vi "Periodic Tasks.vi"(8 "error in":errorcluster) -> ()   [LabVIEW 2018]
doc: "This VI runs in parallel to other tasks. It can contain as many user-defined periodic loops as you need. These can carry out PID or other sorts of timed response."
uses:
  <vilib>/Rock Robotics/WPI/DriverStation/WPI_DriverStationRobotMode2.ctl
  <vilib>/Rock Robotics/WPI/Utilities/WPI_GetSetVariantRefNum.vi
  Robot Global Data.vi
  <vilib>/Rock Robotics/WPI/ThirdParty/Phoenix-LabVIEW/Motor Controller/Get/CTRE_Phoenix_MotorController_GetSelectedSensorData.vi
panel:
  out "Y position":dbl
  out "X position":dbl
  out "status":dbl
  out "Yaw":dbl
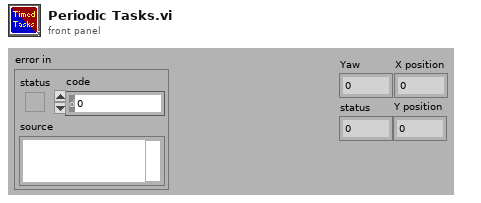
[diagram p1: front panel]
types:
  T1 = typedef "WPI_JoystickDevRef.ctl" = cluster{"Device":T2}
  T2 = typedef "WPI_JoystickDeviceEnum.ctl" = enum16{"USB 0", "USB 1", "USB 2", "USB 3", "USB 4", "USB 5"}
  T3 = typedef "WPI_RobotDriveDevRef.ctl" = cluster{"DevStatus":errorcluster, "Motors[]":T4[], "Square Inputs":bool, "Max Output":dbl}
  T4 = typedef "WPI_MotorControlDeviceRef.ctl" = cluster{"DeviceStatus":errorcluster, "Type":T5, "PWM":cluster{"PWM Channel":T6, "DeadBand":T7}, "CAN":cluster{"Device Number":u8, "SetOutput VI Ref":variant, "GetOutput VI Ref":variant, "Enable VI Ref":variant, "Disable VI Ref":variant, "Data":variant}, "Invert":bool, "DIO PWM":cluster{"PWM \"Enable\" Channel":T6, "DIOChannel":T8, "PWM Rate":dbl}}
  T5 = typedef "WPI_MotorControlType.ctl" = enum16{"PWM", "CAN", "DIO PWM"}
  T6 = typedef "FPGA_DIOPWMChannel.ctl" = enum8{"PWM 0", "PWM 1", "PWM 2", "PWM 3", "PWM 4", "PWM 5", "PWM 6", "PWM 7", "PWM 8", "PWM 9", "PWM MXP 0", "PWM MXP 1", "PWM MXP 2", "PWM MXP 3", "PWM MXP 4", "PWM MXP 5", "PWM MXP 6", "PWM MXP 7", "PWM MXP 8", "PWM MXP 9", "Invalid"}
  T7 = typedef "WPI_PWMDeadband.ctl" = cluster{"Name":string, "maxPositivePwm":i32, "minPositivePwm":i32, "centerPwm":i32, "maxNegativePwm":i32, "minNegativePwm":i32, "angularRange":u16}
  T8 = typedef "FPGA_DIOChannel.ctl" = enum8{"DIO 0", "DIO 1", "DIO 2", "DIO 3", "DIO 4", "DIO 5", "DIO 6", "DIO 7", "DIO 8", "DIO 9", "DIO MXP 0", "DIO MXP 1", "DIO MXP 2", "DIO MXP 3", "DIO MXP 4", "DIO MXP 5", "DIO MXP 6", "DIO MXP 7", "DIO MXP 8", "DIO MXP 9", "DIO MXP 10", "DIO MXP 11", "DIO MXP 12", "DIO MXP 13", "DIO MXP 14", "DIO MXP 15", "SPI Port CS1", "SPI Port CS2", "SPI Port CS3", "SPI Port MISO", "SPI Port MOSI", "Invalid"}
  T9 = cluster{"JoystickDevRef":T1, "RobotDriveDevRef":T3}
  T10 = typedef "WPI_DriverStationRobotMode2.ctl" = enum16{"Autonomous Disabled", "Autonomous Enabled", "Teleop Disabled", "Teleop Enabled", "Disconnected", "Finish", "Test Disabled", "Test Enabled", "Emergency Stopped"}
  T11 = cluster{"Yaw":dbl, "Roll":dbl, "Pitch":dbl, "Heading":dbl, "Fused Heading":dbl}
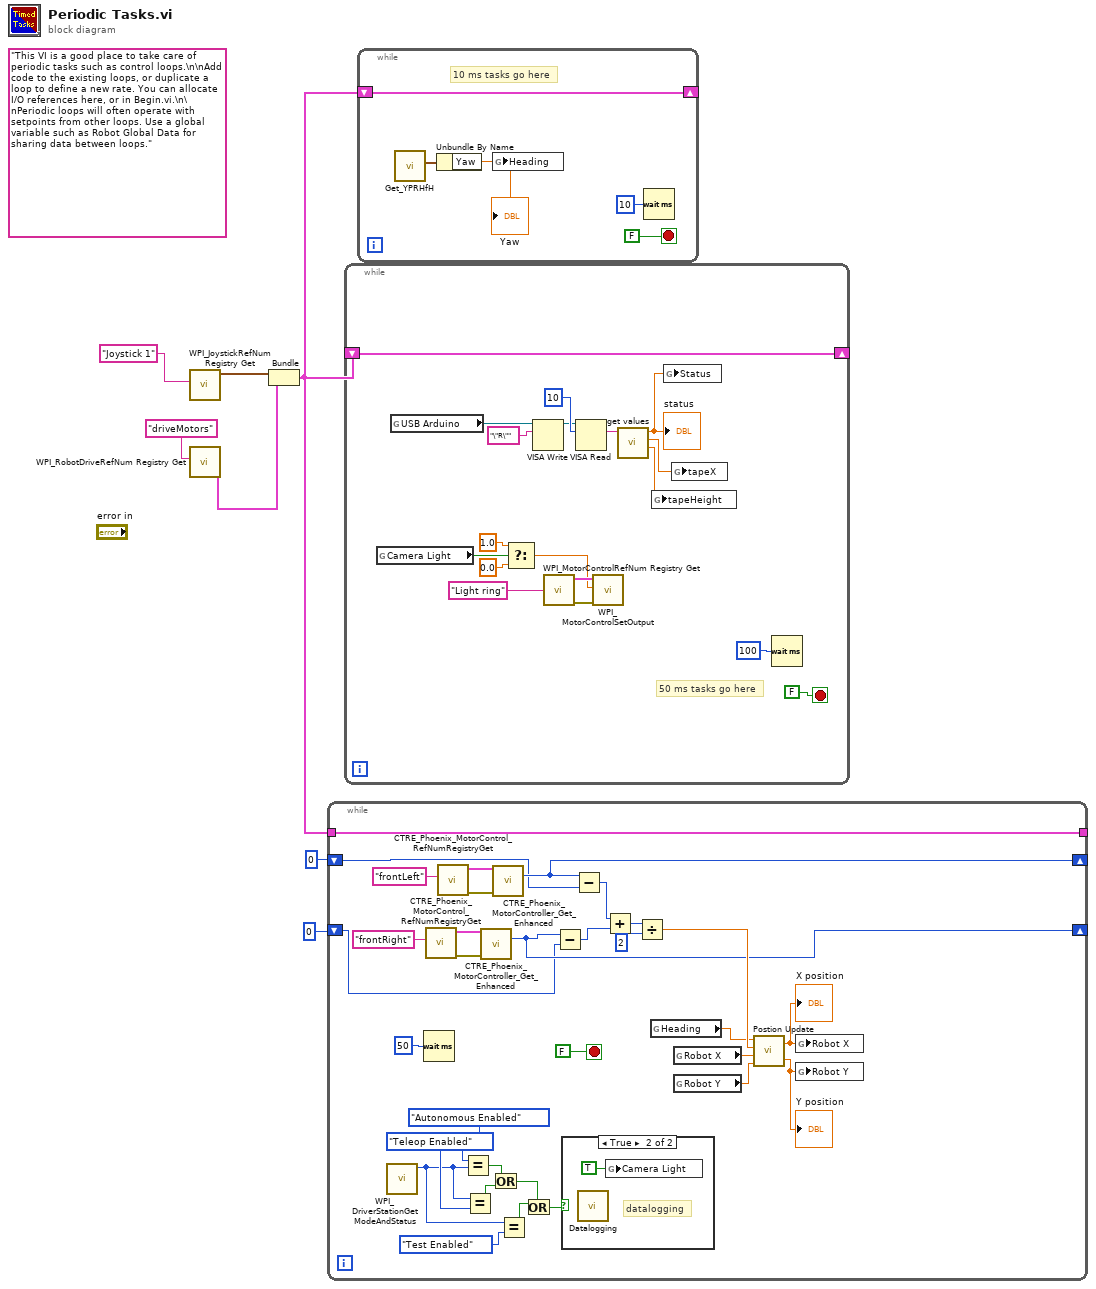
[diagram p0: block diagram]
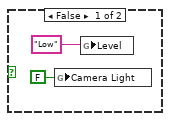
[diagram p2: hidden frame]
diagram:
  (unwired) "This VI is a good place to take care of periodic tasks such as control loops.\n\nAdd code to the existing loops, or duplicate a loop to define a new rate. You can allocate I/O references here, or in Begin.vi.\n\nPeriodic loops will often operate with setpoints from other loops. Use a global variable such as Robot Global Data for sharing data between loops."
  n1 = call <vilib>:"WPI_JoystickRefNum Registry Get.vi"("refnum name"="Joystick 1") -> ("JoystickDevRef"=w5:T1)  [unwired: 1 in, 9 out]
  n2 = call <vilib>:"WPI_RobotDriveRefNum Registry Get.vi"("refnum name"="driveMotors") -> ("RobotDriveDevRef"=w4:T3)  [unwired: 1 in, 9 out]
  n3 = Bundle("JoystickDevRef"=w5, "RobotDriveDevRef"=w4) -> (w3:T9)  [unwired: 1 out]
  n4 = while {
    tunnel: w3 -> [w39]
    tunnel: [w39] -> _
    shift-right: [w22] -> _
    shift-left: 0 -> [w21]
    shift-right: [w20] -> _
    shift-left: 0 -> [w19]
    stop <- FALSE stop-if-true
    n5 = call <vilib>:"WPI_DriverStationGetModeAndStatus.vi"() -> ("Robot Mode"=w12:T10)  [unwired: 10 in, 1 out]
    n6 = Wait (ms)(milliseconds to wait=u32 50) -> ()  [unwired: 1 out]
    n7 = call <vilib>:"CTRE_Phoenix_MotorControl_RefNumRegistryGet.vi"("refnum name"="frontRight") -> ("error out"=w33:errorcluster, "PhoenixMotorControlDevRef"=w31:T4)  [unwired: 9 in]
    n8 = call <vilib>:"CTRE_Phoenix_MotorControl_RefNumRegistryGet.vi"("refnum name"="frontLeft") -> ("error out"=w35:errorcluster, "PhoenixMotorControlDevRef"=w36:T4)  [unwired: 9 in]
    n9 = Equal?(x=WPI_DriverStationRobotMode2."Autonomous Enabled" ("Robot Mode"), y=w12) -> (x = y?=w15:bool)
    n10 = Equal?(x=w12, y=WPI_DriverStationRobotMode2."Teleop Enabled" ("Robot Mode")) -> (x = y?=w9:bool)
    n11 = call-poly <vilib>:"CTRE_Phoenix_MotorController_Get_Enhanced.vi"("PhoenixMotorControlDevRef"=w31, "error in"=w33) -> ("Position (Raw Sensor Units)"=w20:i32)  [unwired: 10 in, 3 out]
    n12 = Or(x=w15, y=w9) -> (x .or. y?=w8:bool)
    n13 = call-poly <vilib>:"CTRE_Phoenix_MotorController_Get_Enhanced.vi"("PhoenixMotorControlDevRef"=w36, "error in"=w35) -> ("Position (Raw Sensor Units)"=w22:i32)  [unwired: 10 in, 3 out]
    n14 = Equal?(x=w12, y=WPI_DriverStationRobotMode2."Test Enabled" ("Robot Mode")) -> (x = y?=w13:bool)
    n15 = Or(x=w13, y=w8) -> (x .or. y?=w10:bool)
    n16 = Subtract(x=w20, y=w19) -> (x-y=w24:i32)
    n17 = case shown="True" w10 {
      frame False {
        n18 = global write "Robot Global Data.vi" "Camera Light"(FALSE ("Camera Light")) -> ()
        n19 = global write "Robot Global Data.vi" "Level"("Low" ("Level")) -> ()
      }
      frame True {
        # "datalogging"
        n20 = call "Datalogging.vi"() -> ()  [unwired: 12 in]
        n21 = global write "Robot Global Data.vi" "Camera Light"(TRUE ("Camera Light")) -> ()
      }
    }
    n22 = Subtract(x=w22, y=w21) -> (x-y=w23:i32)
    n23 = Add(x=w23, y=w24) -> (x+y=w30:i32)
    n24 = Divide(x=w30, y=2) -> (x/y=w28:dbl)
    n25 = global read "Robot Global Data.vi" "Heading"() -> (w27:dbl)
    n26 = global read "Robot Global Data.vi" "Robot X"() -> (w37:dbl)
    n27 = global read "Robot Global Data.vi" "Robot Y"() -> (w38:dbl)
    n28 = call "Postion Update.vi"("Y position in"=w38, "X position in"=w37, "Distance"=w28, "Heading"=w27) -> ("Y position"=w17:dbl, "X position"=w18:dbl)
    "X position" <- w18
    "Y position" <- w17
    n29 = global write "Robot Global Data.vi" "Robot X"(w18) -> ()
    n30 = global write "Robot Global Data.vi" "Robot Y"(w17) -> ()
  }
  n31 = while {
    shift-right: [w58] -> _
    shift-left: w3 -> [w58]
    stop <- FALSE stop-if-true
    # "50 ms tasks go here"
    n32 = global read "Robot Global Data.vi" "Camera Light"() -> (w47:bool)
    n33 = global read "Robot Global Data.vi" "USB Arduino"() -> (w52:refnum<visa-resource-name>)
    n34 = Select(t=1.0, s=w47, f=0.0) -> (s? t:f=w44:dbl)
    n35 = VISA Write(VISA resource name=w52, write buffer="\"R\"") -> (VISA resource name out=w51:refnum<visa-resource-name>)  [unwired: 1 in, 2 out]
    n36 = call <vilib>:"WPI_MotorControlRefNum Registry Get.vi"("refnum name"="Light ring") -> ("error out"=w49:errorcluster, "MotorControlDevRef"=w48:T4)  [unwired: 9 in]
    n37 = VISA Read(VISA resource name=w51, byte count=u32 10) -> (read buffer=w54:string)  [unwired: 1 in, 3 out]
    n38 = call <vilib>:"WPI_MotorControlSetOutput.vi"("error in (no error)"=w49, "Output"=w44, "MotorControlDevRef"=w48) -> ()  [unwired: 6 in, 3 out]
    n39 = call "get values.vi"("USB In"=w54) -> ("insidex (0-319)"=w55:dbl, "averagex (0-319)"=w56:dbl, "status"=w57:dbl)  [unwired: 8 in]
    "status" <- w57
    n40 = global write "Robot Global Data.vi" "tapeHeight"(w55) -> ()
    n41 = global write "Robot Global Data.vi" "Status"(w57) -> ()
    n42 = global write "Robot Global Data.vi" "tapeX"(w56) -> ()
    n43 = Wait (ms)(milliseconds to wait=u32 100) -> ()  [unwired: 1 out]
  }
  n44 = while {
    shift-right: [w63] -> _
    shift-left: w3 -> [w63]
    stop <- FALSE stop-if-true
    # "10 ms tasks go here"
    n45 = call <vilib>:"Get_YPRHfH.vi"() -> ("YRPHfH"=w62:T11)  [unwired: 11 in]
    n46 = Unbundle By Name(w62) -> ("Yaw"=w61:dbl)
    "Yaw" <- w61
    n47 = global write "Robot Global Data.vi" "Heading"(w61) -> ()
    n48 = Wait (ms)(milliseconds to wait=u32 10) -> ()  [unwired: 1 out]
  }
